vi "ArraySearch_BlockFormation_Maxdisplay Modified_VI.vi"(8 "RR number":i32=4, 10 "読み取り配列":string, 11 "Cutted Sample Sequence":string) -> (0 "出力クラスタ 2":T1, 1 "リード方向総合":enum16{"5’→3'", "3'→5'"}(ring), 2 "最長Right Read値":i32, 3 "Right Read MAX":string, 4 "配列終了番号":i32, 5 "R number":i32, 6 "配列開始番号":i32, 7 "元配列数":i32, 9 "重複？":bool)   [LabVIEW 2018]
panel:
  out "逆前削減配列判定マトリクス":bool[][](array[boolean])
  out "順前削減配列判定マトリクス":bool[][](array[boolean])
  out "Good":bool
  out "順削減配列Max No":i32
  out "順前削減配列Max要素":string
  out "逆前削減配列Max No":i32
  out "逆前削減配列Max要素":string
  out "Later Read":string
  out "Right Read":string
  out "Front Read":string
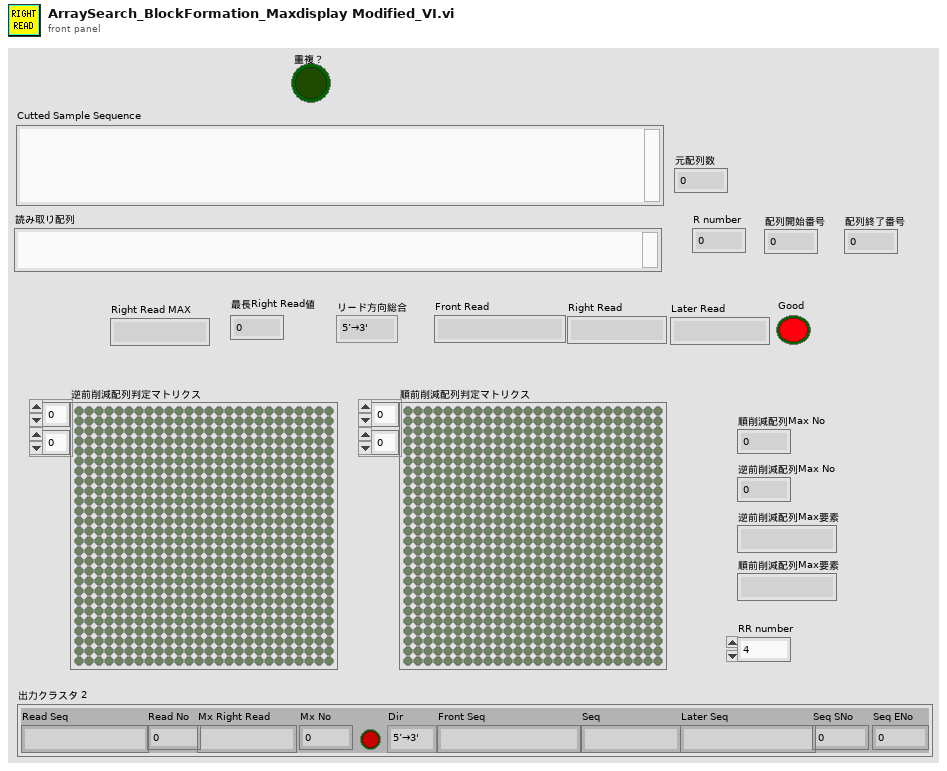
[diagram p1: front panel]
types:
  T1 = cluster{"Read Seq":string, "Read No":i32, "Mx Right Read":string, "Mx No":i32, "Dir":enum16{"5’→3'", "3'→5'"}, "Front Seq":string, "Seq":string, "Later Seq":string, bool, "Seq SNo":i32, "Seq ENo":i32}
  T2 = cluster{"読み取り配列":string, "読み取り長さ":i32, "Right Read MAX":string, "最長Right Read値":i32, "リード方向":enum16{"5’→3'", "3'→5'"}, "Front Read":string, "Right Read":string, "Later Read":string, bool, i32, i32}
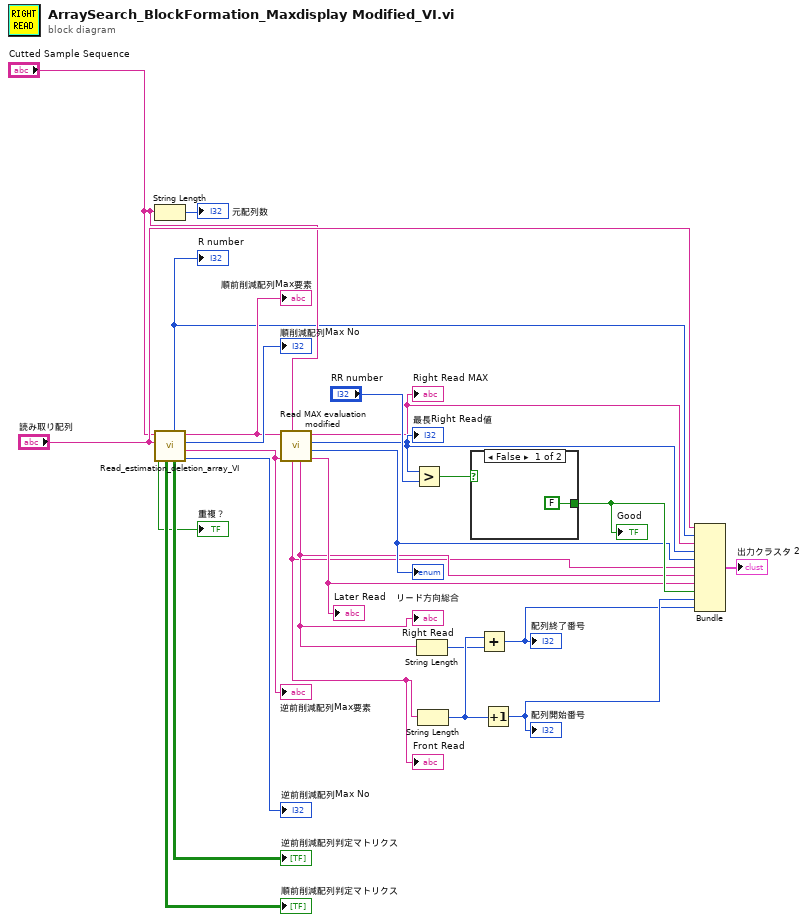
[diagram p0: block diagram]
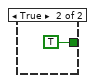
[diagram p2: hidden frame]
diagram:
  n1 = String Length(string="Cutted Sample Sequence") -> (length=→"元配列数":i32)
  n2 = call "Read_estimation_deletion_array_VI.vi"("読み取り配列"="読み取り配列", "元配列"="Cutted Sample Sequence") -> ("逆Maxリード数"=→"逆前削減配列Max No":i32, "逆前削減配列Max Letter X"=w12:string, "順MAXリード数"=→"順削減配列Max No":i32, "順前削減配列 Max L X"=w10:string, "逆前削減配列判定マトリクス"=→"逆前削減配列判定マトリクス":bool[][], "読み取り長さ"=w4:i32, "順前削減配列判定マトリクス"=→"順前削減配列判定マトリクス":bool[][], "重複？"=→"重複？":bool)  [unwired: 1 in, 1 out]
  "R number" <- w4
  "逆前削減配列Max要素" <- w12
  "順前削減配列Max要素" <- w10
  n3 = call "Read MAX evaluation modified.vi"("元配列"="Cutted Sample Sequence", "逆前削減配列Max Letter X"=w12, "順前削減配列 Max L X"=w10) -> ("Later Read"=w8:string, "リード方向"=w9:enum16{"5’→3'", "3'→5'"}, "最長Right Read値"=w13:i32, "Right Read MAX"=w5:string, "Right Read"=w7:string, "Front Read"=w6:string)  [unwired: 3 in]
  "Front Read" <- w6
  "Right Read" <- w7
  "Later Read" <- w8
  "Right Read MAX" <- w5
  "最長Right Read値" <- w13
  "リード方向総合" <- w9
  n4 = Greater?(x=w13, y="RR number") -> (0:w23:bool)
  n5 = String Length(string=w7) -> (length=w19:i32)
  n6 = String Length(string=w6) -> (length=w20:i32)
  n7 = case shown="False" w23 {
    tunnel: [FALSE TRUE] -> w22
    frame False {
    }
    frame True {
    }
  }
  "Good" <- w22
  n8 = Add(x=w20, y=w19) -> (x+y=w17:i32)
  "配列終了番号" <- w17
  n9 = Increment(x=w20) -> (x+1=w18:i32)
  "配列開始番号" <- w18
  n10 = Bundle("読み取り配列"="読み取り配列", "読み取り長さ"=w4, "Right Read MAX"=w5, "最長Right Read値"=w13, "リード方向"=w9, "Front Read"=w6, "Right Read"=w7, "Later Read"=w8, w22, w18, w17) -> (→"出力クラスタ 2":T2)  [unwired: 1 in]
